vi "Server_selection.vi"(8 "error in (no error)":errorcluster) -> (0 "error out":errorcluster, 2 "path 2":path[](array[path]), 3 "server_name_list":string[](array[string]))   [LabVIEW 2018]
panel:
  out "path_string":string[](array[string])
  out "array":string[][](array[string])
  out "text":string
  out "path":path
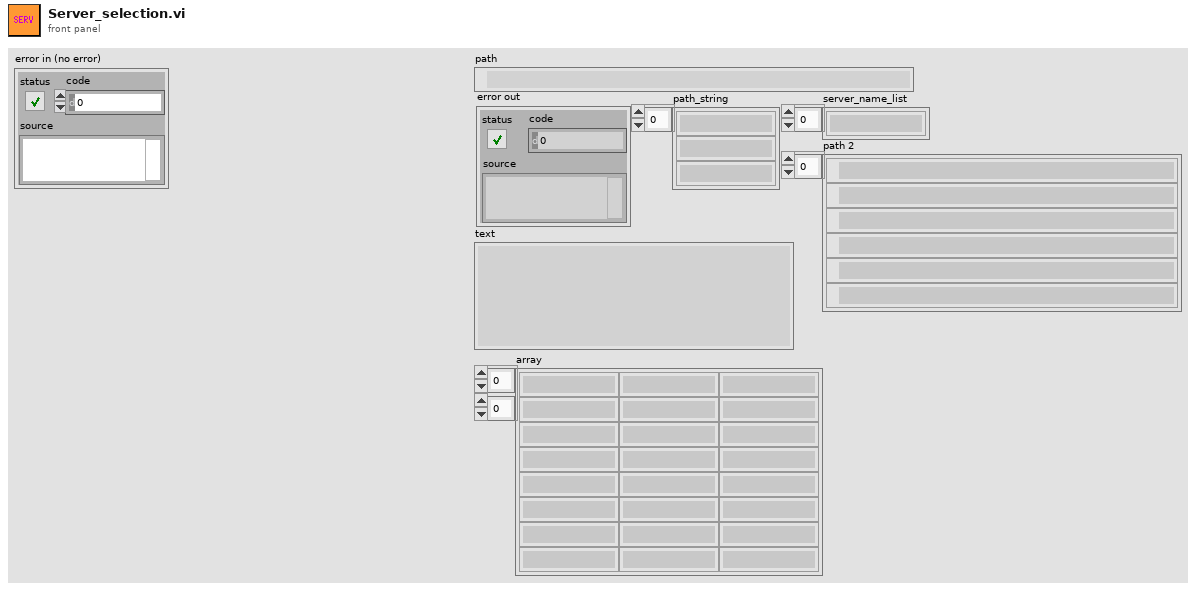
[diagram p1: front panel]
types:
  T1 = enum16{"open", "replace", "create", "open or create", "replace or create", "replace or create with confirmation"}
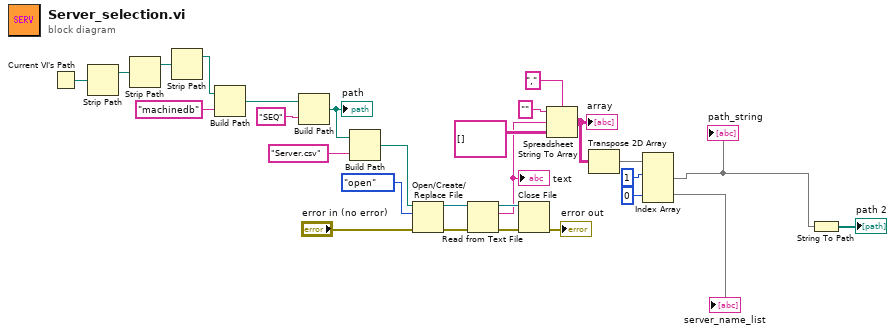
[diagram p0: block diagram]
diagram:
  n1 = Current VI's Path() -> (path=w28:path)
  n2 = Strip Path(path=w28) -> (stripped path=w27:path)  [unwired: 1 out]
  n3 = Strip Path(path=w27) -> (stripped path=w26:path)  [unwired: 1 out]
  n4 = Strip Path(path=w26) -> (stripped path=w25:path)  [unwired: 1 out]
  n5 = Build Path(base path=w25, name or relative path="machinedb") -> (appended path=w23:path)
  n6 = Build Path(base path=w23, name or relative path="SEQ") -> (appended path=w21:path)
  "path" <- w21
  n7 = Build Path(base path=w21, name or relative path="Server.csv") -> (appended path=w17:path)
  n8 = Open/Create/Replace File(file path (use dialog)=w17, error in="error in (no error)", operation (0:open)=T1."open") -> (refnum out=w14:refnum<file>, error out=w19:errorcluster)  [unwired: 3 in, 1 out]
  n9 = Read from Text File(file (use dialog)=w14, error in=w19) -> (refnum out=w13:refnum<file>, text=w10:string, error out=w18:errorcluster)  [unwired: 2 in, 1 out]
  "text" <- w10
  n10 = Close File(refnum=w13, error in=w18) -> (error out=→"error out":errorcluster)  [unwired: 1 out]
  n11 = Spreadsheet String To Array(delimiter (Tab)=",", format string="", spreadsheet string=w10, array type (2D Dbl)=string[][] []) -> (array=w6:string[][])
  "array" <- w6
  n12 = Transpose 2D Array(2D array=w6) -> (transposed array=w5:string[][])
  n13 = Index Array(array=w5, index (row) #1=1 ("index (row)"), index (row) #2=0 ("index (row)")) -> (element #1=w2:string[], element #2=→"server_name_list":string[])  [unwired: 2 in]
  "path_string" <- w2
  n14 = String To Path(string=w2) -> (path=→"path 2":path[])
